vi "Initialize Tasks - 1Task.vi"(6 "initialize and close session behavior":T1, 8 "error in":errorcluster, 11 "session reservation in":refnum<class "Session Reservation.lvclass">) -> (0 "error out":errorcluster, 1 "channel list":string, 2 "task":refnum<class "Session Factory.lvclass">, 3 "session reservation out":refnum<class "Session Reservation.lvclass">)   [LabVIEW 2021, in "Session Management niDAQmx.lvlib"]
doc: "Create the NI-DAQmx driver task from the <b>session reservation in</b>. Returns an error if more than one NI-DAQmx task has been reserved. Use \"Initialize Tasks - NTask.vi\" for multiple tasks."
uses:
  Session Management niDAQmx.lvlib
  <vilib>/Plug-In SDKs/Clients/Session Management V1/Session Reservation/Initialize and Close Session Behavior.ctl
  <vilib>/Plug-In SDKs/Clients/Session Management V1/Session Reservation/Session Reservation.lvclass
  Session Factory/Session Factory.lvclass
  C:/Program Files/National Instruments/LabVIEW 2021/vi.lib/Plug-In SDKs/Sessions/Instrument/ISession Factory/ISession Factory.lvclass
  48a85b3c-9847-4089-941c-2fefb0d6bf24.vi
  <vilib>/Plug-In SDKs/Clients/Session Management V1/Session Reservation/Initialize Sessions with Retry.vi
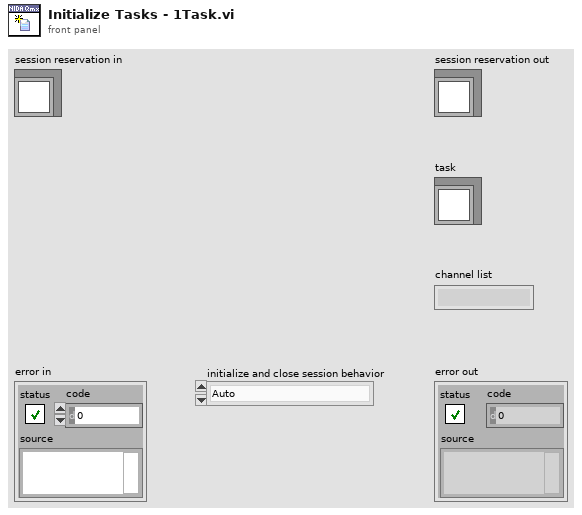
[diagram p1: front panel]
types:
  T1 = typedef "NI Session Management V1 Client.lvlib/Session Reservation.lvclass/Initialize and Close Session Behavior.ctl" = enum16{"Auto", "Initialize and Close", "Attach and Detach", "Initialize and Detach", "Attach and Close"}
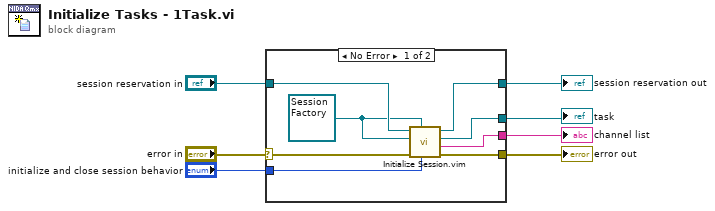
[diagram p0: block diagram]
diagram:
  n1 = case shown="No Error" "error in" {
    selector: "error in" -> [w15 w16]
    tunnel: "session reservation in" -> [w14 w17]
    tunnel: "initialize and close session behavior" -> [w9 _]
    tunnel: [w13 w16] -> w2
    tunnel: [w12 w17] -> w4
    tunnel: [w11 _] -> w1
    tunnel: [w10 _] -> w3
    frame No Error {
      w8 = refnum<class "Session Factory.lvclass"> refnum ("Session Management niDAQmx.lvlib:Session Factory.lvclass")
      n2 = call "Initialize Session.vim"("initialize and close session behavior"=w9, "session type"=w8, "error in"=w15, "session factory"=w8, "session reservation in"=w14) -> ("error out"=w13:errorcluster, "channel list"=w10:string, "session"=w11:refnum<class "Session Factory.lvclass">, "session reservation out"=w12:refnum<class "Session Reservation.lvclass">)  [unwired: 3 in]
    }
    frame Error {
    }
  }
  "error out" <- w2
  "session reservation out" <- w4
  "channel list" <- w3
  "task" <- w1
